vi "SQL_DateTime_SQLstring.vi"(6 "Worltime (f)":bool, 8 "error in (no error)":errorcluster caption="Fehler (Eingang, kein Fehler)") -> (0 "error out":errorcluster caption="Fehler (Ausgang)", 3 "datetime (SQL)":string)   [LabVIEW 2024, in "DB-Tool.lvlib"]
doc: "Get actual Date / Time from PC setting.\n\n<b>Format:</b> YYYY-MM-DD hh:mm:ss\n\nErrorIn have no impact."
uses:
  DB-Tool.lvlib
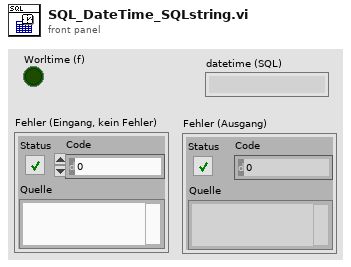
[diagram p1: front panel]
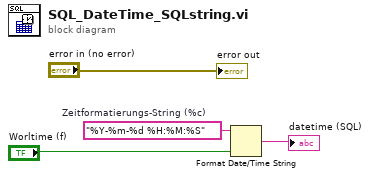
[diagram p0: block diagram]
diagram:
  w4 = "%Y-%m-%d %H:%M:%S"  # Zeitformatierungs-String (%c)
  n1 = Format Date/Time String(time format string (%c)=w4, UTC format="Worltime (f)") -> (date/time string=→"datetime (SQL)":string)  [unwired: 1 in]
  "error out" <- "error in (no error)"
